vi "File_Parsing_Logic.vi"() -> ()   [LabVIEW 2023]
panel:
  out "Array 3":T1(array[cluster])
  out "Array 2":i32[](array[numeric])
  out "Values":T2
  out "GPS Values":T3
  out "result string":string
  in  "File path":path
  out "Array":dbl[](array[numeric])
  in  "Path":path
  # "Row 4"
  # "ROW 0"
  # "Row 2"
  # "Row 4"
  # "Row 1"
  # "Row 5"
  # "Row 3"
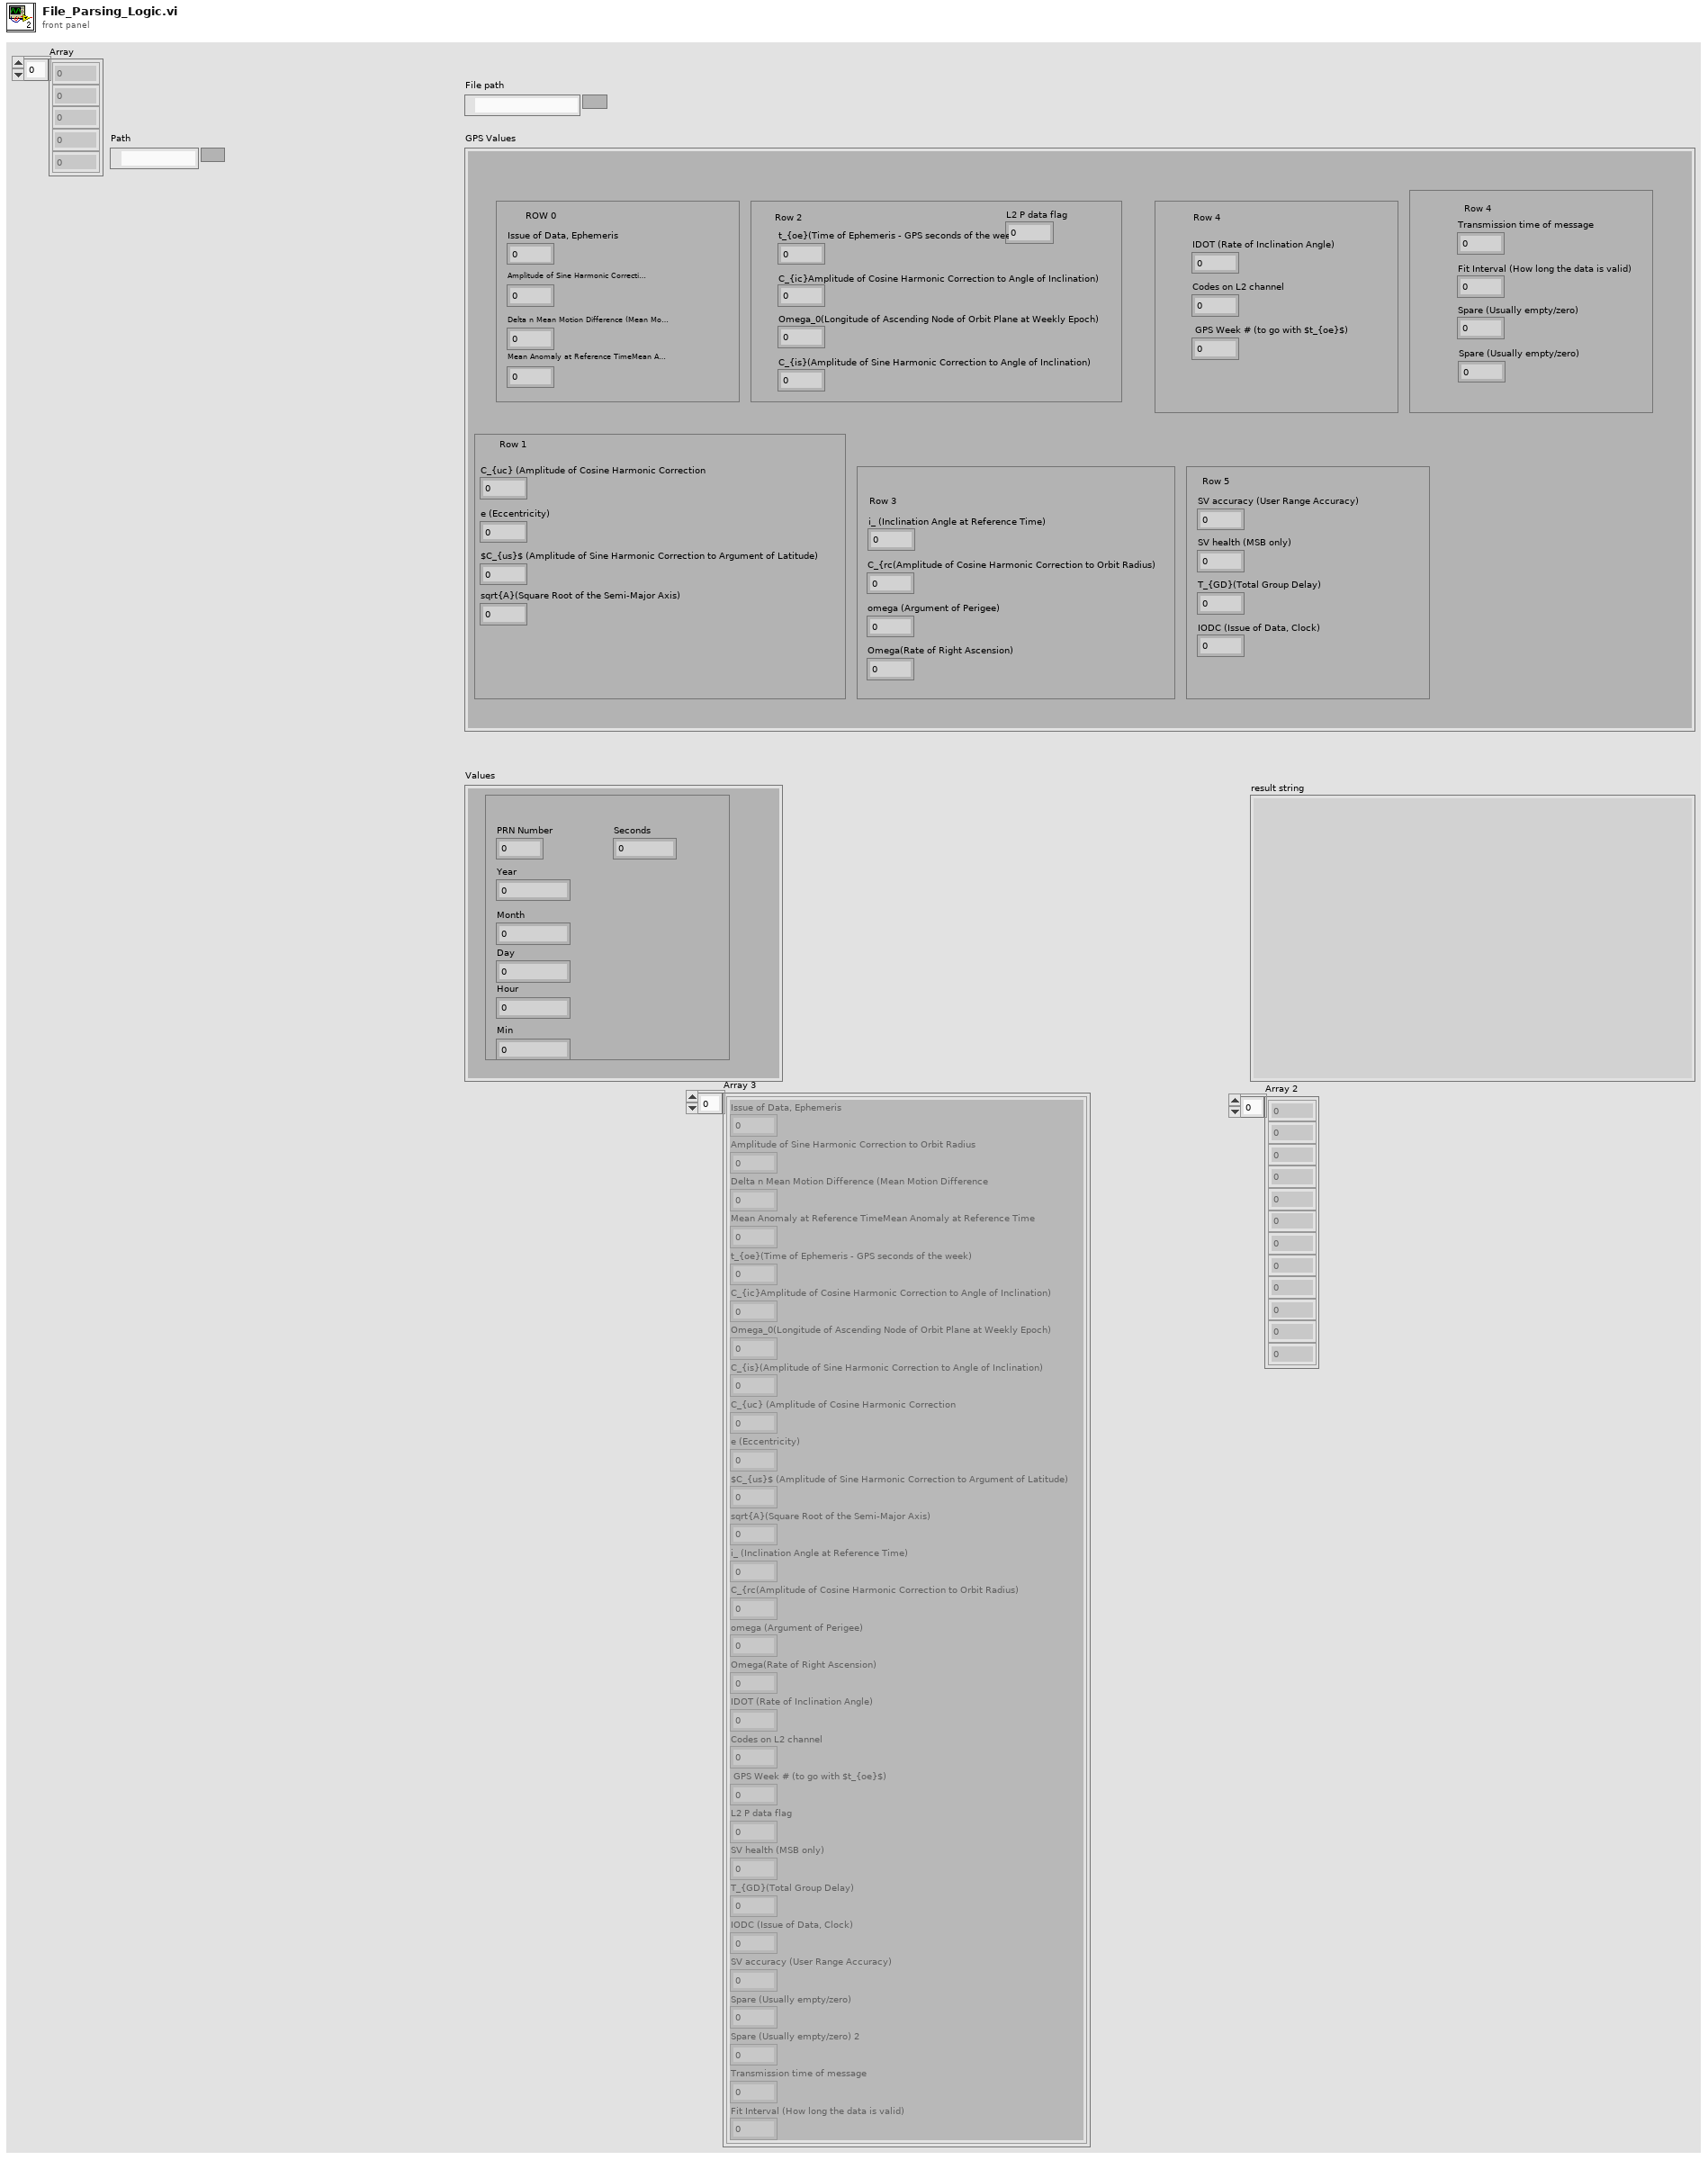
[diagram p1: front panel]
types:
  T1 = cluster{"Issue of Data, Ephemeris":dbl, "Amplitude of Sine Harmonic Correction to Orbit Radius":dbl, "Delta n Mean Motion Difference (Mean Motion Difference":dbl, "Mean Anomaly at Reference TimeMean Anomaly at Reference Time":dbl, "t_{oe}(Time of Ephemeris - GPS seconds of the week)":dbl, "C_{ic}Amplitude of Cosine Harmonic Correction to Angle of Inclination)":dbl, "Omega_0(Longitude of Ascending Node of Orbit Plane at Weekly Epoch)":dbl, "C_{is}(Amplitude of Sine Harmonic Correction to Angle of Inclination)":dbl, "C_{uc} (Amplitude of Cosine Harmonic Correction":dbl, "e (Eccentricity)":dbl, "$C_{us}$ (Amplitude of Sine Harmonic Correction to Argument of Latitude)":dbl, "sqrt{A}(Square Root of the Semi-Major Axis)":dbl, "i_ (Inclination Angle at Reference Time)":dbl, "C_{rc(Amplitude of Cosine Harmonic Correction to Orbit Radius)":dbl, "omega (Argument of Perigee)":dbl, "Omega(Rate of Right Ascension)":dbl, "IDOT (Rate of Inclination Angle)":dbl, "Codes on L2 channel":dbl, " GPS Week # (to go with $t_{oe}$)":dbl, "L2 P data flag":dbl, "SV health (MSB only)":dbl, "T_{GD}(Total Group Delay)":dbl, "IODC (Issue of Data, Clock)":dbl, "SV accuracy (User Range Accuracy)":dbl, "Spare (Usually empty/zero)":dbl, "Spare (Usually empty/zero) 2":dbl, "Transmission time of message":dbl, "Fit Interval (How long the data is valid)":dbl}[]
  T2 = cluster{"PRN Number":dbl, "Year":dbl, "Month":dbl, "Day":dbl, "Hour ":dbl, "Min ":dbl, "Seconds":dbl}
  T3 = cluster{"Issue of Data, Ephemeris":dbl, "Amplitude of Sine Harmonic Correction to Orbit Radius":dbl, "Delta n Mean Motion Difference (Mean Motion Difference":dbl, "Mean Anomaly at Reference TimeMean Anomaly at Reference Time":dbl, "C_{uc} (Amplitude of Cosine Harmonic Correction":dbl, "e (Eccentricity)":dbl, "$C_{us}$ (Amplitude of Sine Harmonic Correction to Argument of Latitude)":dbl, "sqrt{A}(Square Root of the Semi-Major Axis)":dbl, "t_{oe}(Time of Ephemeris - GPS seconds of the week)":dbl, "C_{ic}Amplitude of Cosine Harmonic Correction to Angle of Inclination)":dbl, "Omega_0(Longitude of Ascending Node of Orbit Plane at Weekly Epoch)":dbl, "C_{is}(Amplitude of Sine Harmonic Correction to Angle of Inclination)":dbl, "i_ (Inclination Angle at Reference Time)":dbl, "C_{rc(Amplitude of Cosine Harmonic Correction to Orbit Radius)":dbl, "omega (Argument of Perigee)":dbl, "Omega(Rate of Right Ascension)":dbl, "Spare (Usually empty/zero)":dbl, "Spare (Usually empty/zero)":dbl, "IDOT (Rate of Inclination Angle)":dbl, "Codes on L2 channel":dbl, " GPS Week # (to go with $t_{oe}$)":dbl, "L2 P data flag":dbl, "SV health (MSB only)":dbl, "T_{GD}(Total Group Delay)":dbl, "IODC (Issue of Data, Clock)":dbl, "Transmission time of message":dbl, "Fit Interval (How long the data is valid)":dbl, "SV accuracy (User Range Accuracy)":dbl}
  T4 = cluster{"Issue of Data, Ephemeris":dbl, "Amplitude of Sine Harmonic Correction to Orbit Radius":dbl, "Delta n Mean Motion Difference (Mean Motion Difference":dbl, "Mean Anomaly at Reference TimeMean Anomaly at Reference Time":dbl, "t_{oe}(Time of Ephemeris - GPS seconds of the week)":dbl, "C_{ic}Amplitude of Cosine Harmonic Correction to Angle of Inclination)":dbl, "Omega_0(Longitude of Ascending Node of Orbit Plane at Weekly Epoch)":dbl, "C_{is}(Amplitude of Sine Harmonic Correction to Angle of Inclination)":dbl, "C_{uc} (Amplitude of Cosine Harmonic Correction":dbl, "e (Eccentricity)":dbl, "$C_{us}$ (Amplitude of Sine Harmonic Correction to Argument of Latitude)":dbl, "sqrt{A}(Square Root of the Semi-Major Axis)":dbl, "i_ (Inclination Angle at Reference Time)":dbl, "C_{rc(Amplitude of Cosine Harmonic Correction to Orbit Radius)":dbl, "omega (Argument of Perigee)":dbl, "Omega(Rate of Right Ascension)":dbl, "IDOT (Rate of Inclination Angle)":dbl, "Codes on L2 channel":dbl, " GPS Week # (to go with $t_{oe}$)":dbl, "L2 P data flag":dbl, "SV health (MSB only)":dbl, "T_{GD}(Total Group Delay)":dbl, "IODC (Issue of Data, Clock)":dbl, "SV accuracy (User Range Accuracy)":dbl, "Spare (Usually empty/zero)":dbl, "Spare (Usually empty/zero) 2":dbl, "Transmission time of message":dbl, "Fit Interval (How long the data is valid)":dbl}
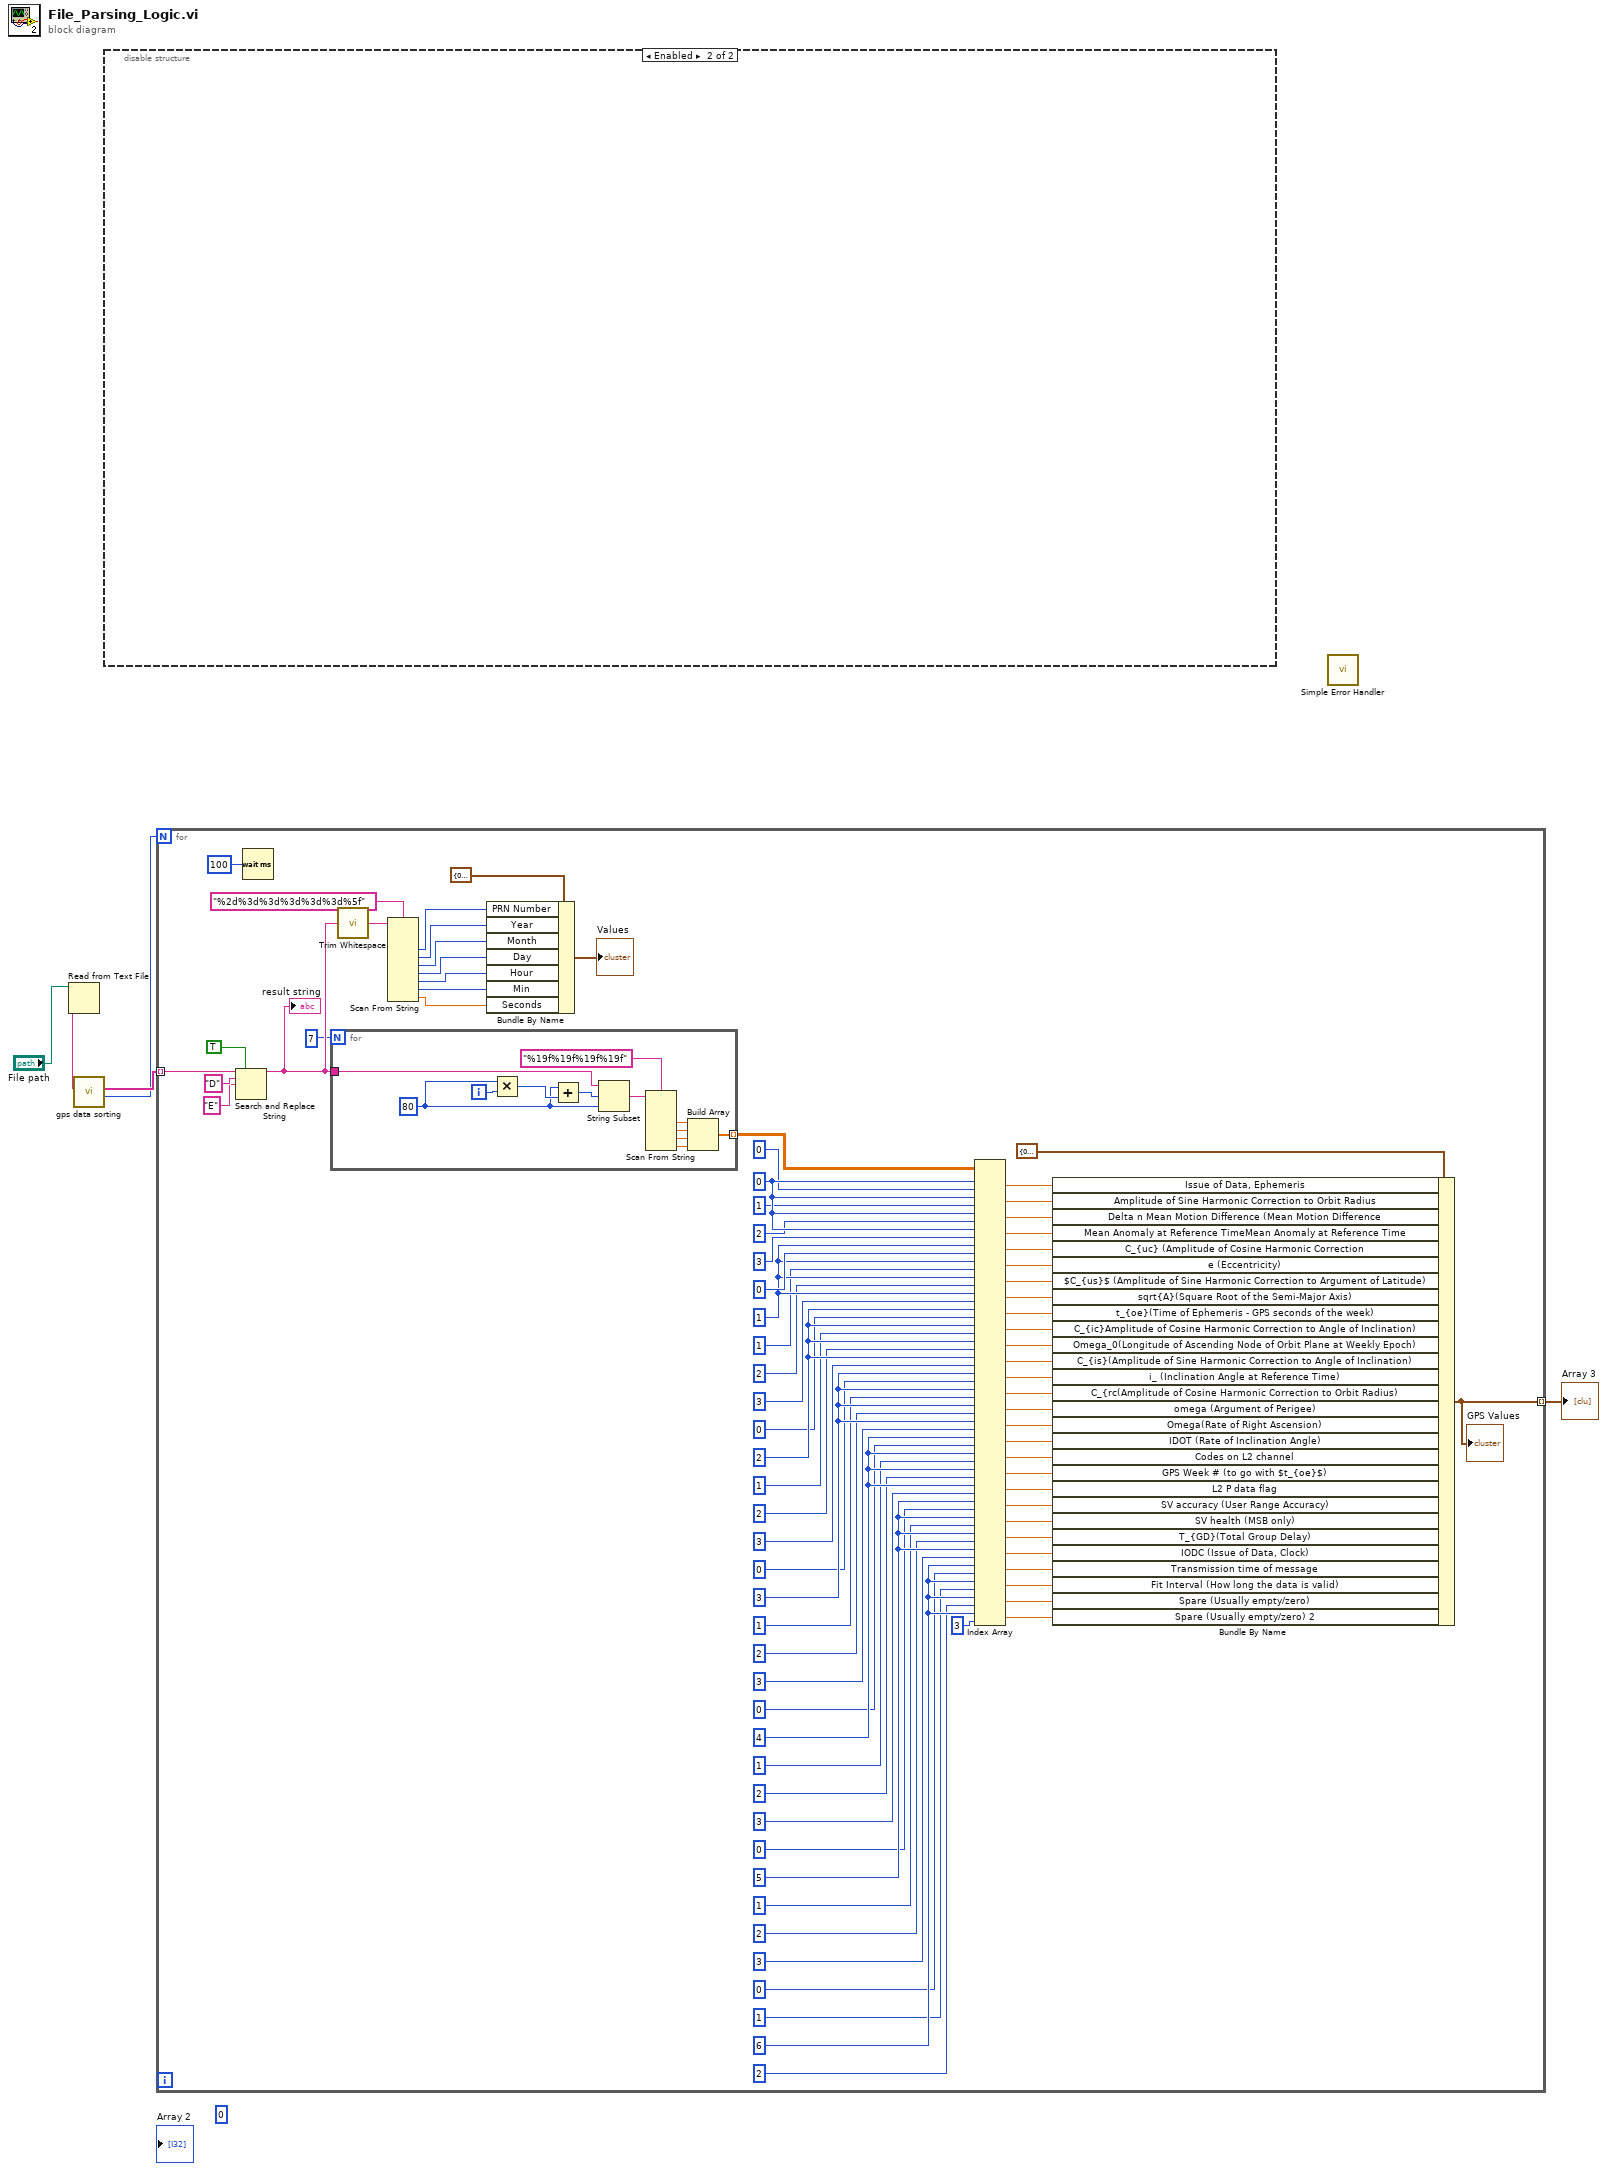
[diagram p0: block diagram]
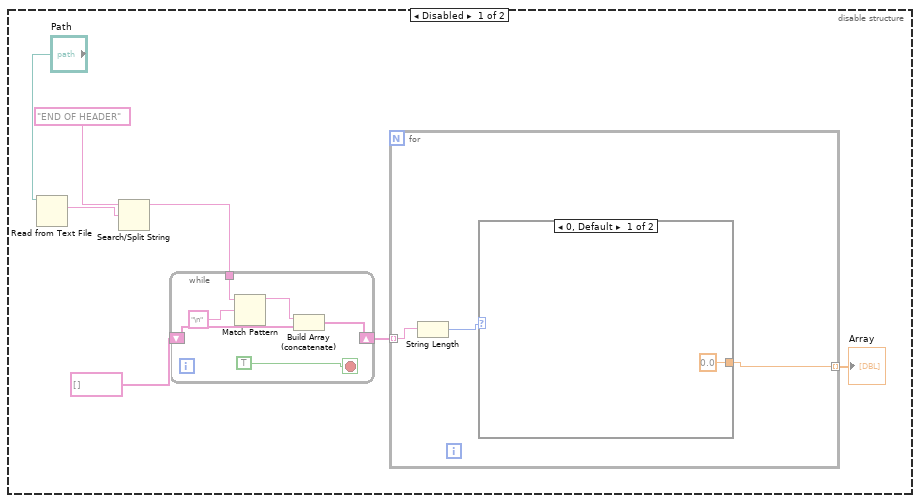
[diagram p2: hidden frame]
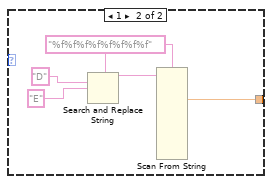
[diagram p3: hidden frame]
diagram:
  (unwired) 0 ("length (rest)")
  n1 = Read from Text File(file (use dialog)="File path") -> (text=w3:string)  [unwired: 3 in, 3 out]
  n2 = call "gps data sorting.vi"("input string"=w3) -> ("unsigned 32bit integer"=w1:u32, "Array 5"=w2:string[])  [unwired: 9 in]
  n3 = disable-structure shown="Enabled" {
    frame Disabled {
      n4 = Read from Text File(file (use dialog)="Path") -> (text=w11:string)  [unwired: 3 in, 3 out]
      n5 = Search/Split String(string="END OF HEADER", search string/char (-)=w11) -> (substring before match=w9:string)  [unwired: 1 in, 2 out]
      n6 = while {
        tunnel: w9 -> [w25]
        shift-right: [w23] -> w7
        shift-left: string[] [] ("Array - String") -> [w22]
        stop <- TRUE ("stop") stop-if-true
        n7 = Match Pattern(string=w25, regular expression="\n") -> (before substring=w24:string)  [unwired: 1 in, 3 out]
        n8 = Build Array (concatenate)(w24, w22) -> (w23:string[])
      }
      n9 = for {
        tunnel: w7 -> [w15] mode=indexing
        tunnel: [w13] -> w6 mode=indexing
        n10 = String Length(string=w15) -> (length=w14:i32)
        n11 = case shown="0, Default" w14 {
          tunnel: [0.0 w19] -> w13
          frame 0, Default {
          }
          frame 1 {
            w17 = "%f%f%f%f%f%f%f%f" ("format string")
            n12 = Search and Replace String(input string=w17, search string="D", replace string="E" ("replace string (\"\")")) -> (result string=w18:string)  [unwired: 5 in, 3 out]
            n13 = Scan From String "Scan From String"(format string=w17, input string=w18) -> (output 1=w19:dbl)  [unwired: 17 in, 3 out]
          }
        }
      }
      "Array" <- w6
    }
    frame Enabled {
    }
  }
  n14 = for {
    N: w1 -> [_]
    tunnel: w2 -> [w28] mode=indexing
    tunnel: [w29] -> w4 mode=indexing
    w73 = 5 ("index (row)")
    w78 = 4 ("index (row)")
    w83 = 3 ("index (row)")
    w88 = 2 ("index (row)")
    w92 = 1 ("index (row)")
    w98 = 0 ("index (row)")
    w104 = 6 ("index (row)")
    n15 = Search and Replace String(replace all?=TRUE ("replace all? (F)"), input string=w28, search string="D", replace string="E" ("replace string (\"\")")) -> (result string=w106:string)  [unwired: 4 in, 3 out]
    "result string" <- w106
    n16 = Wait (ms)(milliseconds to wait=u32 100) -> ()  [unwired: 1 out]
    n17 = for {
      N: 7 -> [_]
      tunnel: w106 -> [w123]
      tunnel: [w112] -> w99 mode=indexing
      i -> [w122]
      w120 = 80 ("length (rest)")
      n18 = Multiply(x=w120, y=w122) -> (x*y=w121:i32)
      n19 = Add(x=w120, y=w121) -> (x+y=w119:i32)
      n20 = String Subset(string=w123, offset (0)=w119, length (rest)=w120) -> (substring=w118:string)
      n21 = Scan From String(format string="%19f%19f%19f%19f", input string=w118) -> (output 1=w116:dbl, output 2=w115:dbl, output 3=w114:dbl, output 4=w113:dbl)  [unwired: 6 in, 3 out]
      n22 = Build Array(w116, w115, w114, w113) -> (w112:dbl[])
    }
    n23 = call <vilib>:"Trim Whitespace.vi"("string"=w106) -> ("trimmed string"=w105:string)  [unwired: 1 in]
    n24 = Scan From String(format string="%2d%3d%3d%3d%3d%3d%5f", input string=w105) -> (output 1=w38:i32, output 2=w37:i32, output 3=w36:i32, output 4=w35:i32, output 5=w34:i32, output 6=w33:i32, output 7=w32:dbl)  [unwired: 9 in, 3 out]
    n25 = Bundle By Name(cluster=T2 {"PRN Number"=0.0, "Year"=0.0, "Month"=0.0, "Day"=0.0, "Hour "=0.0, "Min "=0.0, "Seconds"=0.0} ("input cluster"), "PRN Number"=w38, "Year"=w37, "Month"=w36, "Day"=w35, "Hour"=w34, "Min"=w33, "Seconds"=w32) -> (→"Values":T2)
    n26 = Index Array(array=w99, index (row) #1=w98, index (col) #1=0 ("index (row)"), index (row) #2=w98, index (col) #2=1 ("disabled index (col)"), index (row) #3=w98, index (col) #3=2 ("index (row)"), index (row) #4=w98, index (col) #4=3 ("index (row)"), index (row) #5=w92, index (col) #5=0 ("index (row)"), index (row) #6=w92, index (col) #6=1 ("disabled index (col)"), index (row) #7=w92, index (col) #7=2 ("index (row)"), index (row) #8=w92, index (col) #8=3 ("index (row)"), index (row) #9=w88, index (col) #9=0 ("index (row)"), index (row) #10=w88, index (col) #10=1 ("disabled index (col)"), index (row) #11=w88, index (col) #11=2 ("index (row)"), index (row) #12=w88, index (col) #12=3 ("index (row)"), index (row) #13=w83, index (col) #13=0 ("index (row)"), index (row) #14=w83, index (col) #14=1 ("disabled index (col)"), index (row) #15=w83, index (col) #15=2 ("index (row)"), index (row) #16=w83, index (col) #16=3 ("index (row)"), index (row) #17=w78, index (col) #17=0 ("index (row)"), index (row) #18=w78, index (col) #18=1 ("disabled index (col)"), index (row) #19=w78, index (col) #19=2 ("index (row)"), index (row) #20=w78, index (col) #20=3 ("index (row)"), index (row) #21=w73, index (col) #21=0 ("index (row)"), index (row) #22=w73, index (col) #22=1 ("disabled index (col)"), index (row) #23=w73, index (col) #23=2 ("index (row)"), index (row) #24=w73, index (col) #24=3 ("index (row)"), index (row) #25=w104, index (col) #25=0 ("index (row)"), index (row) #26=w104, index (col) #26=1 ("disabled index (col)"), index (row) #27=w104, index (col) #27=2 ("index (row)"), index (row) #28=w104, index (col) #28=3 ("index (row)")) -> (element #1=w67:dbl, element #2=w66:dbl, element #3=w65:dbl, element #4=w64:dbl, element #5=w63:dbl, element #6=w62:dbl, element #7=w61:dbl, element #8=w60:dbl, element #9=w59:dbl, element #10=w58:dbl, element #11=w57:dbl, element #12=w56:dbl, element #13=w55:dbl, element #14=w54:dbl, element #15=w53:dbl, element #16=w52:dbl, element #17=w51:dbl, element #18=w50:dbl, element #19=w49:dbl, element #20=w48:dbl, element #21=w47:dbl, element #22=w46:dbl, element #23=w45:dbl, element #24=w44:dbl, element #25=w42:dbl, element #26=w41:dbl, element #27=w40:dbl, element #28=w39:dbl)
    n27 = Bundle By Name(cluster=T4 {"Issue of Data, Ephemeris"=0.0, "Amplitude of Sine Harmonic Correction to Orbit Radius"=0.0, "Delta n Mean Motion Difference (Mean Motion Difference"=0.0, "Mean Anomaly at Reference TimeMean Anomaly at Reference Time"=0.0, "t_{oe}(Time of Ephemeris - GPS seconds of the week)"=0.0, "C_{ic}Amplitude of Cosine Harmonic Correction to Angle of Inclination)"=0.0, "Omega_0(Longitude of Ascending Node of Orbit Plane at Weekly Epoch)"=0.0, "C_{is}(Amplitude of Sine Harmonic Correction to Angle of Inclination)"=0.0, "C_{uc} (Amplitude of Cosine Harmonic Correction"=0.0, "e (Eccentricity)"=0.0, "$C_{us}$ (Amplitude of Sine Harmonic Correction to Argument of Latitude)"=0.0, "sqrt{A}(Square Root of the Semi-Major Axis)"=0.0, "i_ (Inclination Angle at Reference Time)"=0.0, "C_{rc(Amplitude of Cosine Harmonic Correction to Orbit Radius)"=0.0, "omega (Argument of Perigee)"=0.0, "Omega(Rate of Right Ascension)"=0.0, "IDOT (Rate of Inclination Angle)"=0.0, "Codes on L2 channel"=0.0, " GPS Week # (to go with $t_{oe}$)"=0.0, "L2 P data flag"=0.0, "SV health (MSB only)"=0.0, "T_{GD}(Total Group Delay)"=0.0, "IODC (Issue of Data, Clock)"=0.0, "SV accuracy (User Range Accuracy)"=0.0, "Spare (Usually empty/zero)"=0.0, "Spare (Usually empty/zero) 2"=0.0, "Transmission time of message"=0.0, "Fit Interval (How long the data is valid)"=0.0} ("input cluster"), "Issue of Data, Ephemeris"=w67, "Amplitude of Sine Harmonic Correction to Orbit Radius"=w66, "Delta n Mean Motion Difference (Mean Motion Difference"=w65, "Mean Anomaly at Reference TimeMean Anomaly at Reference Time"=w64, "C_{uc} (Amplitude of Cosine Harmonic Correction"=w63, "e (Eccentricity)"=w62, "$C_{us}$ (Amplitude of Sine Harmonic Correction to Argument of Latitude)"=w61, "sqrt{A}(Square Root of the Semi-Major Axis)"=w60, "t_{oe}(Time of Ephemeris - GPS seconds of the week)"=w59, "C_{ic}Amplitude of Cosine Harmonic Correction to Angle of Inclination)"=w58, "Omega_0(Longitude of Ascending Node of Orbit Plane at Weekly Epoch)"=w57, "C_{is}(Amplitude of Sine Harmonic Correction to Angle of Inclination)"=w56, "i_ (Inclination Angle at Reference Time)"=w55, "C_{rc(Amplitude of Cosine Harmonic Correction to Orbit Radius)"=w54, "omega (Argument of Perigee)"=w53, "Omega(Rate of Right Ascension)"=w52, "IDOT (Rate of Inclination Angle)"=w51, "Codes on L2 channel"=w50, "GPS Week # (to go with $t_{oe}$)"=w49, "L2 P data flag"=w48, "SV accuracy (User Range Accuracy)"=w47, "SV health (MSB only)"=w46, "T_{GD}(Total Group Delay)"=w45, "IODC (Issue of Data, Clock)"=w44, "Transmission time of message"=w42, "Fit Interval (How long the data is valid)"=w41, "Spare (Usually empty/zero)"=w40, "Spare (Usually empty/zero) 2"=w39) -> (w29:T4)
    "GPS Values" <- w29
  }
  "Array 3" <- w4
  n28 = call <vilib>:"Simple Error Handler.vi"() -> ()  [unwired: 5 in, 5 out]
